vi "Restore AO Outputs.vi"(8 "error in (no error)":errorcluster, 9 "Saved Offsets":dbl[](array[numeric]), 10 "Saved Amplitudes":dbl[](array[numeric]), 11 "Instrument.DAQ in":refnum<class "Instrument.DAQ.lvclass">) -> (0 "error out":errorcluster, 3 "Instrument.DAQ out":refnum<class "Instrument.DAQ.lvclass">)   [LabVIEW 2019, in "Instrument.Lockin.lvlib" / "Instrument.DAQ.lvclass"]
uses:
  Instrument.DAQ.lvclass
  Instrument.DAQ.lvclass/Instrument.DAQ.ctl
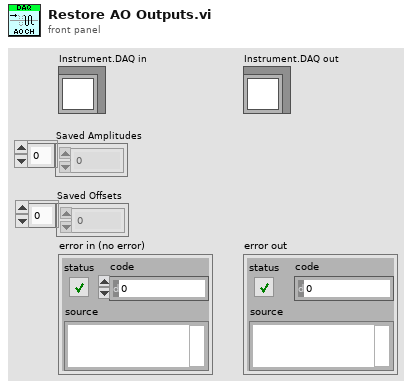
[diagram p1: front panel]
types:
  T1 = typedef "Lockin.Typedefs.lvlib/AO.Channel--Cluster--Array.ctl" = T2[]
  T2 = typedef "Lockin.Typedefs.lvlib/AO.Channel--Cluster.ctl" = cluster{"Enable?":bool, "Channel":i32, "Amplitude":dbl, "Offset":dbl, "Frequency":dbl, "Phase":dbl, "Function":T3, "Sweeping?":bool, "Limit AC":bool, "Limit DC?":bool, "Duty Cycle":bool}
  T3 = typedef "Lockin.Typedefs.lvlib/AO.Channel.Function--Enum.ctl" = enum16{"sine", "square", "triangle", "saw"}
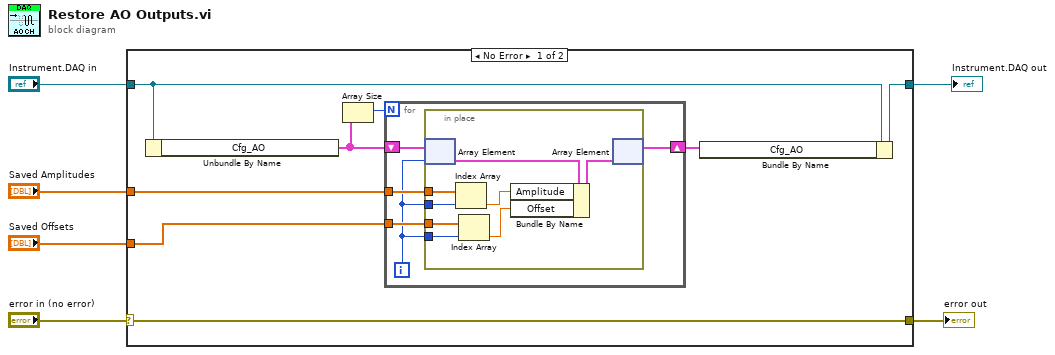
[diagram p0: block diagram]
diagram:
  n1 = case shown="No Error" "error in (no error)" {
    selector: "error in (no error)" -> [w9 w29]
    tunnel: [w13 w28] -> w6
    tunnel: "Instrument.DAQ in" -> [w12 w28]
    tunnel: [w9 w29] -> w3
    tunnel: "Saved Amplitudes" -> [w8 _]
    tunnel: "Saved Offsets" -> [w7 _]
    frame No Error {
      n2 = Unbundle By Name(w12) -> ("Cfg_AO"=w11:T1)
      n3 = Array Size(array=w11) -> (size(s)=w10:i32)
      n4 = for {
        N: w10 -> [_]
        shift-right: [w18] -> w14
        shift-left: w11 -> [w19]
        tunnel: w8 -> [w17]
        tunnel: w7 -> [w16]
        i -> [w15]
        n5 = in-place {
          in-place-border: w17 -> [w24]
          in-place-border: w15 -> [w25]
          in-place-border: w16 -> [w22]
          in-place-border: w15 -> [w20]
          n6 = in-place-array #1(w19, w15) -> (w27:T2)
          n7 = Index Array(array=w24, index=w25) -> (element=w23:dbl)
          n8 = Index Array(array=w22, index=w20) -> (element=w21:dbl)
          n9 = Bundle By Name(cluster=w27, "Amplitude"=w23, "Offset"=w21) -> (w26:T2)
          n10 = in-place-array #1(w26) -> (w18:T1)  [unwired: 1 out]
        }
      }
      n11 = Bundle By Name(cluster=w12, "Cfg_AO"=w14) -> (w13:refnum<class "Instrument.DAQ.lvclass">)
    }
    frame Error {
    }
  }
  "error out" <- w3
  "Instrument.DAQ out" <- w6
